vi "Append Multiple Waveforms.vi"(8 "error in (no error)":errorcluster, 10 "Waveform B []":waveform(dbl)[](array[waveform]), 11 "Waveforrm A []":waveform(dbl)[](array[waveform])) -> (0 "error out":errorcluster, 3 "Waveform out []":waveform(dbl)[](array[waveform]))   [LabVIEW 2019, in "Generator.lvclass"]
uses:
  Generator.lvclass
  <vilib>/Waveform/WDTOps.llb/WDT Append Waveforms DBL.vi
  <vilib>/Waveform/WDTOps.llb/WDT Number of Waveform Samples DBL.vi
panel:
  out "number of samples":i32[](array[numeric])
  out "size(s)":i32
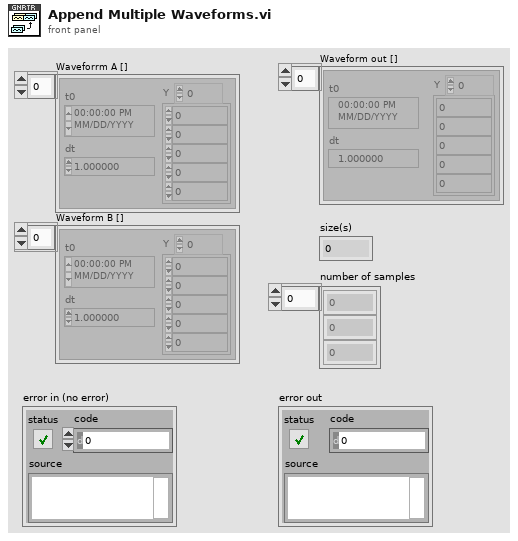
[diagram p1: front panel]
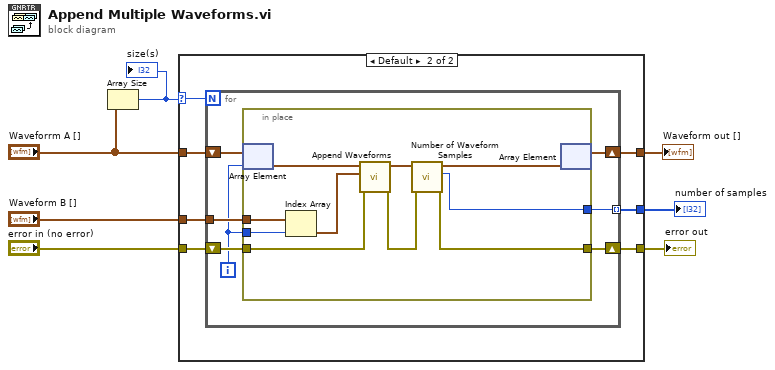
[diagram p0: block diagram]
diagram:
  n1 = Array Size(array="Waveforrm A []") -> (size(s)=w3:i32)
  "size(s)" <- w3
  n2 = case shown="0" w3 {
    selector: w3 -> [_ w11]
    tunnel: [w9 w16] -> w7
    tunnel: "error in (no error)" -> [w8 w15]
    tunnel: "Waveforrm A []" -> [_ w14]
    tunnel: "Waveform B []" -> [w9 w13]
    tunnel: [w8 w12] -> w4
    tunnel: [_ w10] -> w1
    frame 0 {
    }
    frame Default {
      n3 = for {
        N: w11 -> [_]
        tunnel: w13 -> [w21]
        shift-right: [w19] -> w16
        shift-left: w14 -> [w20]
        shift-right: [w22] -> w12
        shift-left: w15 -> [w23]
        tunnel: [w17] -> w10 mode=indexing
        i -> [w18]
        n4 = in-place {
          in-place-border: w23 -> [w29]
          in-place-border: [w27] -> w22
          in-place-border: w21 -> [w33]
          in-place-border: w18 -> [w31]
          in-place-border: [w24] -> w17
          n5 = in-place-array #1(w20, w18) -> (w30:waveform(dbl))
          n6 = Index Array(array=w33, index=w31) -> (element=w32:waveform(dbl))
          n7 = call-poly <vilib>:"Append Waveforms.vi"("error in (no error)"=w29, "waveform B"=w32, "waveform A"=w30) -> ("error out"=w28:errorcluster, "waveform out"=w26:waveform(dbl))  [unwired: 7 in]
          n8 = call-poly <vilib>:"Number of Waveform Samples.vi"("error in (no error)"=w28, "waveform in"=w26) -> ("error out"=w27:errorcluster, "number of samples"=w24:i32, "waveform out"=w25:waveform(dbl))  [unwired: 7 in]
          n9 = in-place-array #1(w25) -> (w19:waveform(dbl)[])  [unwired: 1 out]
        }
      }
    }
  }
  "error out" <- w4
  "Waveform out []" <- w7
  "number of samples" <- w1
